vi "ValueSignalRing.vi"(0 "Ctl Refnum In":refnum<vi>, 5 "Value":string, 11 "Error In":errorcluster) -> (4 "Ctl Refnum Out":refnum<vi>, 15 "Error Out":errorcluster)   [LabVIEW 2019, in "Drona.lvlib"]
doc: "This VI value signals to ring control based on name"
uses:
  Drona.lvlib
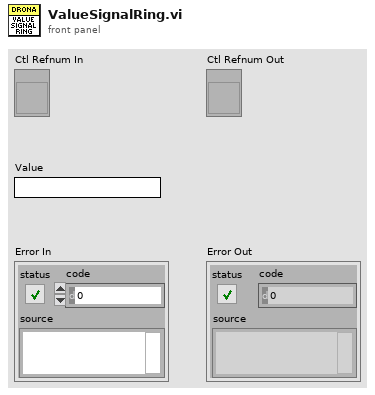
[diagram p1: front panel]
types:
  T1 = typedef "LVStringsAndValuesArrayTypeDef.ctl" = cluster{"String":string, "Value":ext}[]
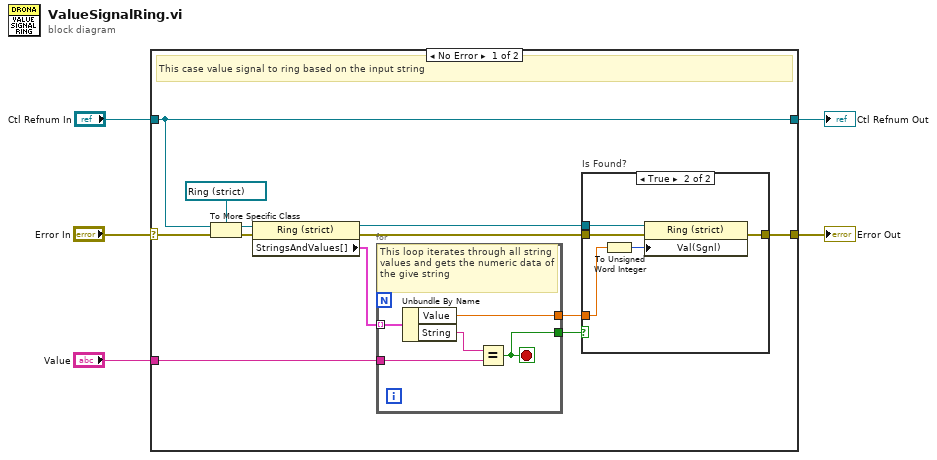
[diagram p0: block diagram]
diagram:
  n1 = case shown="No Error" "Error In" {
    selector: "Error In" -> [w17 w29]
    tunnel: "Ctl Refnum In" -> [w10 w30]
    tunnel: "Value" -> [w14 _]
    tunnel: [w12 w29] -> w2
    tunnel: [w10 w30] -> w1
    frame No Error {
      # "This case value signal to ring based on the input string"
      n2 = To More Specific Class(target class=refnum<vi> refnum ("Ring"), reference=w10, error in=w17) -> (specific class reference=w8:refnum<vi>, error out=w16:errorcluster)
      n3 = property class="Ring (strict)"(reference=w8, error in=w16) -> (reference out=w7:refnum<vi>, error out=w13:errorcluster, "StringsAndValues[]"=w15:T1)
      n4 = for {
        tunnel: w15 -> [w26] mode=indexing
        tunnel: w14 -> [w28]
        tunnel: [w27] -> w11
        tunnel: [w24] -> w6
        stop <- w27 stop-if-true
        # "This loop iterates through all string values and gets the numeric data of the give string"
        n5 = Unbundle By Name(w26) -> ("Value"=w24:ext, "String"=w25:string)
        n6 = Equal?(x=w25, y=w28) -> (x = y?=w27:bool)
      }
      n7 = case "Is Found?" shown="True" w11 {
        tunnel: w13 -> [w18 w23]
        tunnel: [w18 w22] -> w12
        tunnel: w7 -> [_ w21]
        tunnel: w6 -> [_ w20]
        frame False {
        }
        frame True {
          n8 = To Unsigned Word Integer(number=w20) -> (unsigned 16bit integer=w19:u16)
          n9 = property class="Ring (strict)"(reference=w21, error in=w23, "Val(Sgnl)"=w19) -> (error out=w22:errorcluster)  [unwired: 1 out]
        }
      }
    }
    frame Error {
      # "If error, this case pass that error message only"
    }
  }
  "Error Out" <- w2
  "Ctl Refnum Out" <- w1
